vi "Popup_Check_ACK.vi"(8 "error in (no error)":errorcluster={"status"=FALSE, "code"=0, "source"="\"\""}, 10 "Host ACK":string, 11 "Popup state":string) -> (0 "error out":errorcluster={"status"=FALSE, "code"=0, "source"="\"\""}, 2 "status ok":bool, 3 "Pending/acknowledged/timeout":string)   [LabVIEW 2026]
doc: "INTENT: Evaluate ACK combinations. LOGIC: Match request ID/run ID; combine operator/time/feedback conditions per configured AND/OR rule."
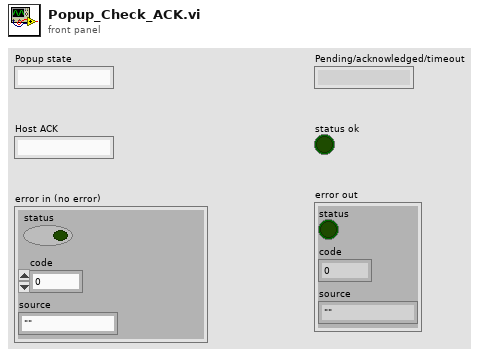
[diagram p1: front panel]
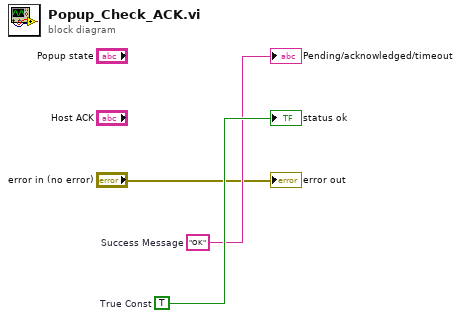
[diagram p0: block diagram]
diagram:
  w3 = TRUE  # True Const
  w2 = "OK"  # Success Message
  "Pending/acknowledged/timeout" <- w2
  "status ok" <- w3
  "error out" <- "error in (no error)"
